vi "FlatToRichauth_StartLoginResponse.vi"(5 "OutputClusterType":T1, 11 "InputCluster":T2) -> (3 "OutputCluster":T1)   [LabVIEW 2020, in "grpc-auth_client.lvlib"]
uses:
  grpc-auth_client.lvlib
  auth_StartLoginResponse_Flat.ctl
  auth_StartLoginResponse.ctl
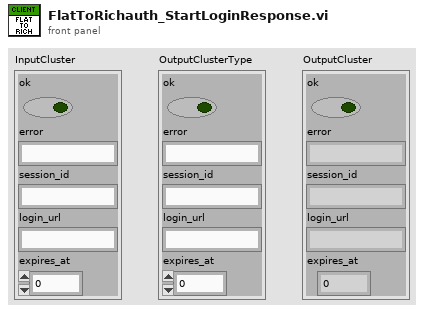
[diagram p1: front panel]
types:
  T1 = typedef "grpc-auth_client.lvlib/auth_StartLoginResponse.ctl" = cluster{"ok":bool, "error":string, "session_id":string, "login_url":string, "expires_at":i64}
  T2 = typedef "grpc-auth_client.lvlib/auth_StartLoginResponse_Flat.ctl" = cluster{"ok":bool, "error":string, "session_id":string, "login_url":string, "expires_at":i64}
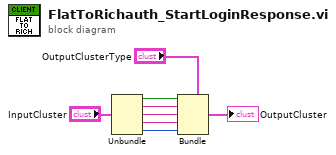
[diagram p0: block diagram]
diagram:
  n1 = Unbundle "Unbundle"("InputCluster") -> ("ok"=w5:bool, "error"=w4:string, "session_id"=w3:string, "login_url"=w2:string, "expires_at"=w1:i64)
  n2 = Bundle "Bundle"(cluster="OutputClusterType", "ok"=w5, "error"=w4, "session_id"=w3, "login_url"=w2, "expires_at"=w1) -> (→"OutputCluster":T1)
